vi "apply_clahe_planar.vi"(4 "clip_limit":sgl=2.0, 8 "error in (no error)":errorcluster, 9 "tile_grid_h":i32=8, 10 "tile_grid_w":i32=8, 11 "image in":T1) -> (0 "error out":errorcluster, 3 "image out":T1)   [LabVIEW 2017, in "Image Processing Library.lvlib"]
uses:
  Image Processing Library.lvlib
  <vilib>/picture/picture.llb/imagedata.ctl
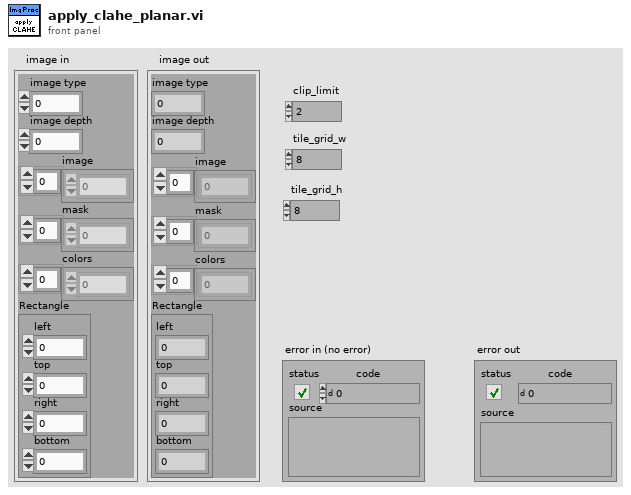
[diagram p1: front panel]
types:
  T1 = typedef "imagedata.ctl" = cluster{"image type":i32, "image depth":i32, "image":u8[], "mask":u8[], "colors":u32[], "Rectangle":cluster{"left":i16, "top":i16, "right":i16, "bottom":i16}}
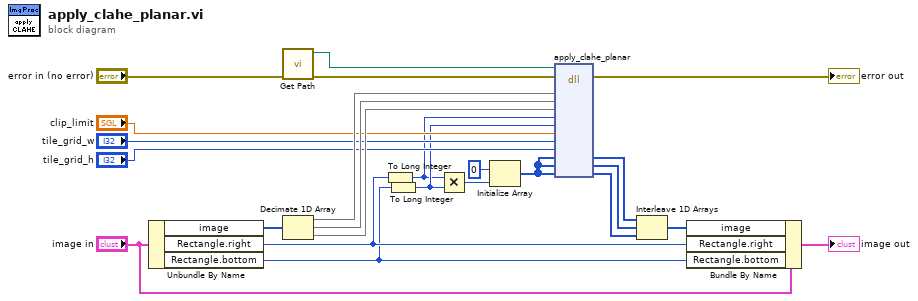
[diagram p0: block diagram]
diagram:
  n1 = Unbundle By Name("image in") -> ("image"=w17:u8[], "Rectangle.right"=w4:i16, "Rectangle.bottom"=w3:i16)
  n2 = call "Get Path.vi"("error in (no error)"="error in (no error)") -> ("error out"=w23:errorcluster, "Library Path"=w22:path)  [unwired: 9 in]
  n3 = Decimate 1D Array(w17) -> (w16:u8[], w15:u8[], w14:u8[])
  n4 = To Long Integer(number=w4) -> (32bit integer=w1:i32)
  n5 = To Long Integer(number=w3) -> (32bit integer=w2:i32)
  n6 = Multiply(x=w1, y=w2) -> (x*y=w20:i32)
  n7 = Initialize Array(u8 0 ("element"), w20) -> (w18:u8[])
  n8 = dll-call lib="C:/Users/IvanLis-Win10/Desktop/LabVIEW/Coin Detector/Project_2018/image_processing/windows_x64/image_processing.dll" fn="apply_clahe_planar"(path in=w22, error in=w23, "in_r"=w16, "in_g"=w15, "in_b"=w14, "orig_w"=w1, "orig_h"=w2, "clip_limit"="clip_limit", "tile_grid_w"="tile_grid_w", "tile_grid_h"="tile_grid_h", "out_r"=w18, "out_g"=w18, "out_b"=w18) -> (error out=→"error out":errorcluster, "out_r"=w13:u8[], "out_g"=w12:u8[], "out_b"=w11:u8[])  [unwired: 10 in, 1 out]
  n9 = Interleave 1D Arrays(w13, w12, w11) -> (w10:u8[])
  n10 = Bundle By Name(cluster="image in", "image"=w10, "Rectangle.right"=w4, "Rectangle.bottom"=w3) -> (→"image out":T1)
